vi "Get Webdav.vi"(8 "error in (no error)":errorcluster, 10 "relative uri":string, 11 "Refnum in":T2) -> (0 "error out":errorcluster, 2 "file list":T1[](array[typedef]) caption="Dateiliste", 3 "session handle out":T2)   [LabVIEW 2020, in "SEECD System Explorer.lvlib"]
uses:
  SEECD System Explorer.lvlib
  <vilib>/WebDAVClient/Advanced/SessionHandle.ctl
  <vilib>/WebDAVClient/Advanced/FileInfo.ctl
  <vilib>/WebDAVClient/NI_WebDAV.lvlib
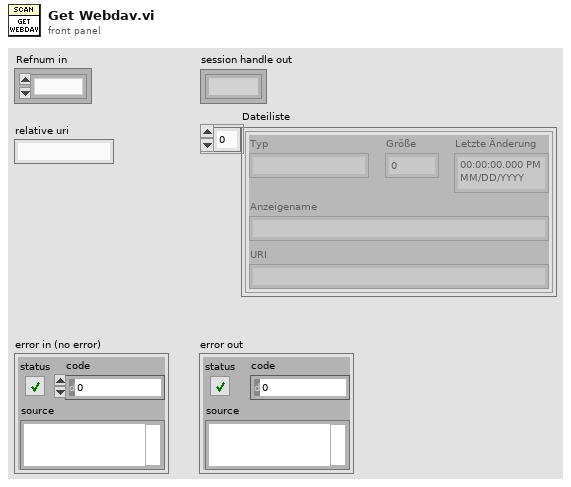
[diagram p1: front panel]
types:
  T1 = typedef "NI_WebDAV.lvlib/FileInfo.ctl" = cluster{"type":string, "size":u64, "last modification":timestamp, "display name":string, "uri":string}
  T2 = typedef "NI_WebDAV.lvlib/SessionHandle.ctl" = refnum<k1>
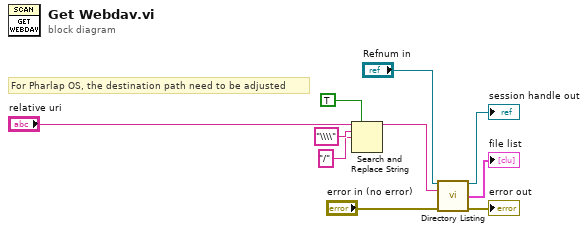
[diagram p0: block diagram]
diagram:
  # "For Pharlap OS, the destination path need to be adjusted"
  n1 = Search and Replace String(replace all?=TRUE ("replace all? (F)"), input string="relative uri", search string="\\\\", replace string="/" ("replace string (\"\")")) -> (result string=w2:string)  [unwired: 4 in, 3 out]
  n2 = call <vilib>:"Directory Listing.vi"("session handle"="Refnum in", "relative uri"=w2, "error in (no error)"="error in (no error)") -> ("session handle out"=→"session handle out":T2, "file list"=→"file list":T1[], "error out"=→"error out":errorcluster)  [unwired: 9 in, 1 out]
